vi "Open.vi"(8 "error in (no error)":errorcluster, 11 "channel in":refnum<class "CANsub_DirectChannel.lvclass">) -> (0 "error out":errorcluster, 3 "channel out":refnum<class "CANsub_DirectChannel.lvclass">)   [LabVIEW 2021, in "CANsub_API.lvlib" / "CANsub_DirectChannel.lvclass"]
doc: "Direct: with an error in, does nothing. Else checks the library version (= 1.2.0, else 5204), opens the channel (C2 before_ws, C4 TLS + Nagle off, C6 handshake, C2 after_ws: accept-all filters), allocates the decoder state and the TX buffer (W12); state = Open. On an error inside Open: C7 cleanup, state stays Closed, the first error is reported. \n\nSetup/teardown only: do not call in a periodic loop (allocates, may block)."
uses:
  CANsub_DirectChannel.lvclass
  CANsub_DirectChannel.lvclass/CANsub_DirectChannel.ctl
  CANsub_C.lvlib
  common/CANsub_Common.lvlib
  common/Typedefs/REST_Phase.ctl
  C_RX_State.ctl
  Typedefs/CANsub_State.ctl
  CANsub_API.lvlib
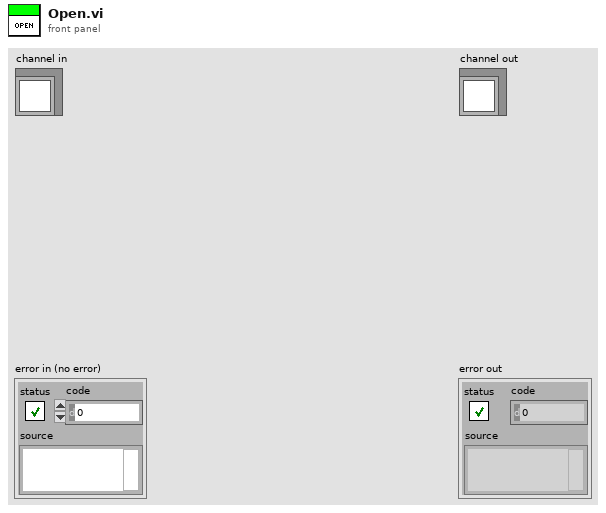
[diagram p1: front panel]
types:
  T1 = typedef "CANsub_Common.lvlib/REST_Phase.ctl" = enum16{"before_ws", "after_ws"}
  T2 = typedef "CANsub_API.lvlib/CANsub_State.ctl" = enum16{"Closed", "Open", "Lost"}
  T3 = typedef "CANsub_C.lvlib/C_RX_State.ctl" = cluster{"ws":u8[], "hdlc":u8[], "ping":u8[]}
  T4 = typedef "CANsub_C.lvlib/C_Info.ctl" = cluster{"version":u32, "hdlc state size":i32, "ws state size":i32, "max frames (4096)":i32}
  T5 = typedef "CANsub_Common.lvlib/Bit_Timing.ctl" = cluster{"brp":u16, "seg1":u16, "seg2":u16, "sjw":u16, "data brp":u16, "data seg1":u16, "data seg2":u16, "data sjw":u16}
  T6 = typedef "CANsub_C.lvlib/C_RX_Buffers.ctl" = cluster{"t_dev":dbl[], "ws":u8[], "id":u32[], "flags":u16[], "hdlc":u8[], "dlc":u8[], "data len":u8[], "data":u8[], "ping":u8[]}
  T7 = typedef "CANsub_API.lvlib/CANsub_Status.ctl" = cluster{"state":T2, "frames read":u32, "frames written":u32, "crc errors":u32, "decode errors":i32, "pings":u32, "FIFO overflows":u32, "reopens":u32, "nodelay":i32, "api version":string, "lib version":u32, "bit timing":T5, "last error":errorcluster}
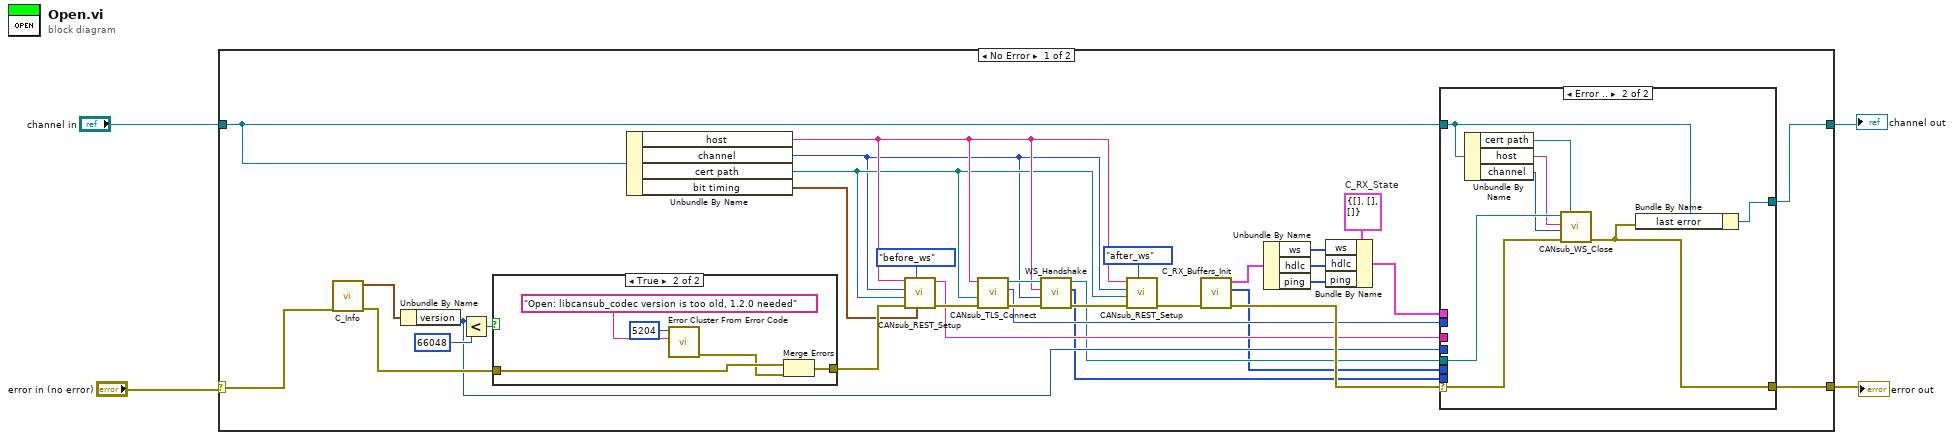
[diagram p0: block diagram]
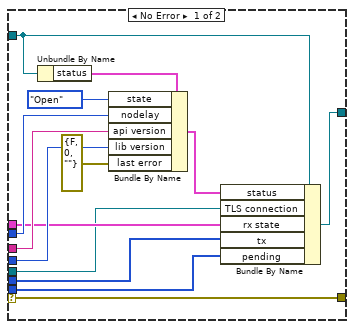
[diagram p2: hidden frame]
diagram:
  n1 = case shown="No Error" "error in (no error)" {
    selector: "error in (no error)" -> [w28 w66]
    tunnel: [w16 w67] -> w3
    tunnel: "channel in" -> [w15 w67]
    tunnel: [w30 w66] -> w1
    frame No Error {
      w20 = T3 {"ws"=[], "hdlc"=[], "ping"=[]}  # C_RX_State
      n2 = call "C_Info.vi"("error in (no error)"=w28) -> ("error out"=w34:errorcluster, "C_Info"=w37:T4)  [unwired: 9 in]
      n3 = Unbundle By Name(w37) -> ("version"=w12:u32)
      n4 = Less?(x=w12, y=u32 66048) -> (x < y?=w35:bool)
      n5 = case shown="True" w35 {
        tunnel: [w60 w63] -> w33
        tunnel: w34 -> [w60 w62]
        frame False {
        }
        frame True {
          n6 = call <vilib>:"Error Cluster From Error Code.vi"("error message (\"\")"="Open: libcansub_codec version is too old, 1.2.0 needed" ("error message (\"\")"), "error code (0)"=5204) -> ("error out"=w61:errorcluster)  [unwired: 7 in]
          n7 = Merge Errors(w62, w61) -> (w63:errorcluster)
        }
      }
      n8 = Unbundle By Name(w15) -> ("host"=w7:string, "channel"=w5:u8, "cert path"=w6:path, "bit timing"=w27:T5)
      n9 = call "CANsub_REST_Setup.vi"("bit timing"=w27, "phase"=REST_Phase."before_ws", "error in (no error)"=w33, "cert path"=w6, "channel"=w5, "host"=w7) -> ("error out"=w32:errorcluster, "api version"=w14:string)  [unwired: 4 in]
      n10 = call "CANsub_TLS_Connect.vi"("error in (no error)"=w32, "cert path"=w6, "host"=w7) -> ("error out"=w25:errorcluster, "nodelay"=w13:i32, "TLS connection"=w22:refnum<k5>)  [unwired: 6 in]
      n11 = call "WS_Handshake.vi"("error in (no error)"=w25, "channel"=w5, "host"=w7, "TLS connection"=w22) -> ("error out"=w24:errorcluster, "leftover"=w8:u8[], "TLS connection out"=w11:refnum<k5>)  [unwired: 4 in, 1 out]
      n12 = call "CANsub_REST_Setup.vi"("phase"=REST_Phase."after_ws", "error in (no error)"=w24, "cert path"=w6, "channel"=w5, "host"=w7) -> ("error out"=w23:errorcluster)  [unwired: 5 in, 1 out]
      n13 = call "C_RX_Buffers_Init.vi"("error in (no error)"=w23) -> ("error out"=w31:errorcluster, "tx"=w9:u8[], "buffers"=w21:T6)  [unwired: 7 in, 1 out]
      n14 = Unbundle By Name(w21) -> ("ws"=w19:u8[], "hdlc"=w18:u8[], "ping"=w17:u8[])
      n15 = Bundle By Name(cluster=w20, "ws"=w19, "hdlc"=w18, "ping"=w17) -> (w10:T3)
      n16 = case shown="Error .." w31 {
        selector: w31 -> [w48 w59]
        tunnel: [w48 w53] -> w30
        tunnel: [w49 w52] -> w16
        tunnel: w15 -> [w46 w54]
        tunnel: w14 -> [w43 _]
        tunnel: w13 -> [w44 _]
        tunnel: w12 -> [w42 _]
        tunnel: w11 -> [w40 w58]
        tunnel: w10 -> [w41 _]
        tunnel: w9 -> [w39 _]
        tunnel: w8 -> [w38 _]
        frame No Error {
          n17 = Unbundle By Name(w46) -> ("status"=w47:T7)
          n18 = Bundle By Name(cluster=w47, "state"=CANsub_State."Open" ("status.state"), "nodelay"=w44, "api version"=w43, "lib version"=w42, "last error"=errorcluster {"status"=FALSE, "code"=0, "source"=""} ("status.last error")) -> (w45:T7)
          n19 = Bundle By Name(cluster=w46, "status"=w45, "TLS connection"=w40, "rx state"=w41, "tx"=w39, "pending"=w38) -> (w49:refnum<class "CANsub_DirectChannel.lvclass">)
        }
        frame Error {
          n20 = Unbundle By Name(w54) -> ("cert path"=w57:path, "host"=w56:string, "channel"=w55:u8)
          n21 = call "CANsub_WS_Close.vi"("cert path"=w57, "error in (no error)"=w59, "channel"=w55, "host"=w56, "TLS Connection"=w58) -> ("error out"=w53:errorcluster)  [unwired: 5 in, 1 out]
          n22 = Bundle By Name(cluster=w54, "last error"=w53) -> (w52:refnum<class "CANsub_DirectChannel.lvclass">)
        }
      }
    }
    frame Error {
    }
  }
  "error out" <- w1
  "channel out" <- w3
